vi "constant_jdp_pgsql.vi"() -> (0 "jdp_pgsql_mapper":refnum<class "Mapper.lvclass">, 1 "jdp_pgsql_dbc":refnum<class "DBC.lvclass">)   [LabVIEW 2020, in "ORM_API_jdp.lvlib"]
uses:
  <vilib>/Viviota/shared/ORM_pgsql_jdp.lvlibp/dbc/DBC.lvclass
  <vilib>/Viviota/shared/ORM_pgsql_jdp.lvlibp/PGJDPMapper/Mapper.lvclass
  ORM_API_jdp.lvlib
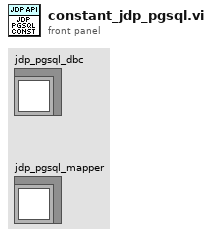
[diagram p1: front panel]
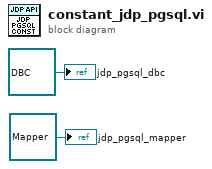
[diagram p0: block diagram]
diagram:
  "jdp_pgsql_dbc" <- refnum<class "DBC.lvclass"> refnum ("ORM_pgsql_jdp.lvlibp:DBC.lvclass")
  "jdp_pgsql_mapper" <- refnum<class "Mapper.lvclass"> refnum ("ORM_pgsql_jdp.lvlibp:Mapper.lvclass")
